vi "VIH ProjFile - Path Converter - Write.vi"(11 "Path in":path) -> (3 "Path out":path)   [LabVIEW 2014]
doc: "::: VI Helpeks :::\nCopyright (c) 2000-2026 Konstantin Shifershteyn. All rights reserved."
panel:
  # "VI Helpeks\nCopyright (c) 2012-2026 Konstantin Shifershteyn"
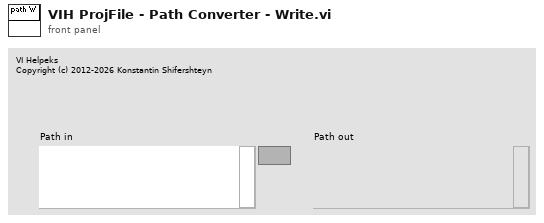
[diagram p1: front panel]
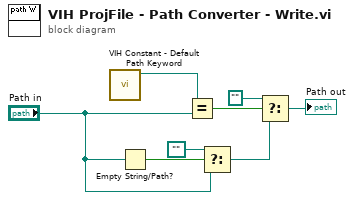
[diagram p0: block diagram]
diagram:
  n1 = call "VIH Constant - Default Path Keyword.vi"() -> ("<default> path"=w1:path)  [unwired: 11 in]
  n2 = Empty String/Path?(string/path="Path in") -> (empty?=w7:bool)
  n3 = Equal?(x=w1, y="Path in") -> (x = y?=w5:bool)
  n4 = Select(t=path "" ("y"), s=w7, f="Path in") -> (s? t:f=w6:path)
  n5 = Select(t=path "", s=w5, f=w6) -> (s? t:f=→"Path out":path)
